vi "RemoteVI Copy Window.vi"(0 "hwnd":u64, 11 "error in":errorcluster) -> (4 "pixmap":u32[][](array[numeric]), 15 "error out":errorcluster)   [LabVIEW 2020, in "RemoteVI.lvlib"]
doc: "Copies the CLIENT AREA of the window hwnd into a 2D U32 pixmap [row, column] of 0x00RRGGBB values as Windows composited it last: user32 GetDC of the window, gdi32 BitBlt (SRCCOPY) into a memory bitmap of the client size (user32 GetClientRect), GetDIBits as 32-bit top-down rows. With desktop composition every top-level window draws into its own surface, so this sees the window's pixels whether or not it is covered by other windows (measured on Windows 11 with a LabVIEW front panel behind a maximised window, pixel-identical to PrintWindow) - and unlike PrintWindow it does not make the window draw itself again: about 2-5 ms for an 817 x 543 panel instead of 40-50 ms with PrintWindow, during which LabVIEW's UI thread repainted the whole window (graph included) for every frame and was busy for nothing else (measured on the demo). A minimized window has an empty client area; pixmap is then empty. No VI Server call, so it works while an open popup holds LabVIEW's UI thread. Every GDI object is deselected and released again, also when an earlier step failed. error out carries error in, a Call Library Function Node error, 5003 when BitBlt failed or 5001 when GetDIBits copied no line."
uses:
  RemoteVI.lvlib
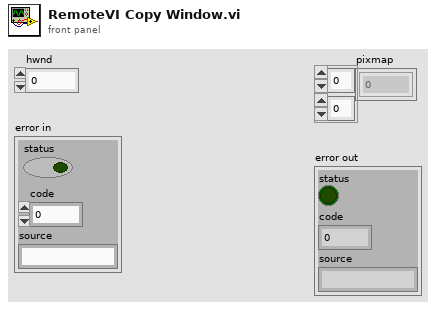
[diagram p1: front panel]
types:
  T1 = cluster{"left":i32, "top":i32, "right":i32, "bottom":i32}
  T2 = cluster{"biSize":u32, "right":i32, i32, "biPlanes":u16, "biBitCount":u16, u32, u32, "zero":i32, "zero":i32, u32, u32, u32}
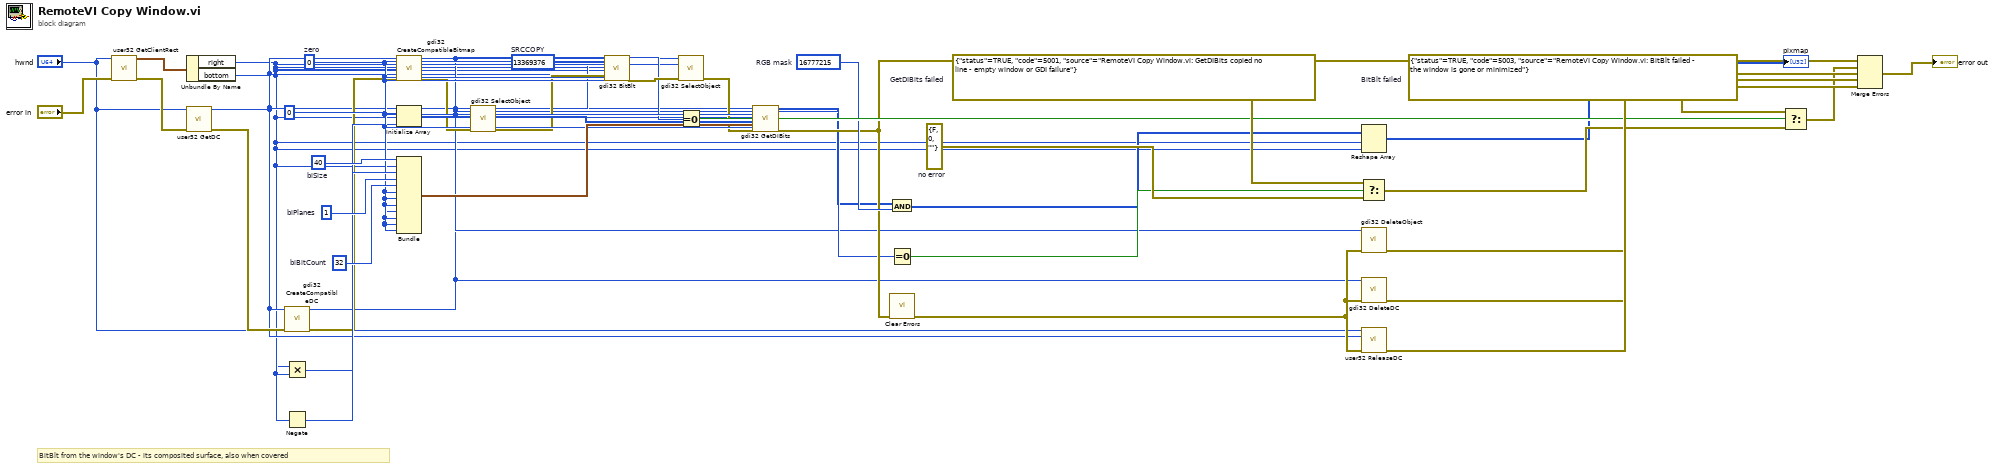
[diagram p0: block diagram]
diagram:
  w39 = errorcluster {"status"=FALSE, "code"=0, "source"=""}  # no error
  w38 = errorcluster {"status"=TRUE, "code"=5001, "source"="RemoteVI Copy Window.vi: GetDIBits copied no line - empty window or GDI failure"}  # GetDIBits failed
  w37 = errorcluster {"status"=TRUE, "code"=5003, "source"="RemoteVI Copy Window.vi: BitBlt failed - the window is gone or minimized"}  # BitBlt failed
  w33 = u32 16777215  # RGB mask
  w28 = u16 32  # biBitCount
  w27 = u16 1  # biPlanes
  w26 = u32 40  # biSize
  w23 = u32 0
  w18 = u32 13369376  # SRCCOPY
  w17 = 0  # zero
  # "BitBlt from the window's DC - its composited surface, also when covered"
  n1 = call "user32 GetClientRect.vi"("hWnd"="hwnd", "error in"="error in") -> ("RECT"=w5:T1, "error out"=w6:errorcluster)  [unwired: 11 in, 1 out]
  n2 = Unbundle By Name(w5) -> ("right"=w7:i32, "bottom"=w8:i32)
  n3 = call "user32 GetDC.vi"("hWnd"="hwnd", "error in"=w6) -> ("HDC"=w9:u64, "error out"=w10:errorcluster)  [unwired: 12 in]
  n4 = call "gdi32 CreateCompatibleDC.vi"("hdc"=w9, "error in"=w10) -> ("HDC"=w11:u64, "error out"=w12:errorcluster)  [unwired: 12 in]
  n5 = Multiply(x=w7, y=w8) -> (x*y=w22:i32)
  n6 = Negate(x=w8) -> (-x=w25:i32)
  n7 = call "gdi32 CreateCompatibleBitmap.vi"("hdc"=w9, "cx"=w7, "cy"=w8, "error in"=w12) -> ("HBITMAP"=w13:u64, "error out"=w14:errorcluster)  [unwired: 10 in]
  n8 = Initialize Array(w23, w22) -> (w24:u32[])
  n9 = Bundle("biSize"=w26, "right"=w7, w25, "biPlanes"=w27, "biBitCount"=w28, w23, w23, "zero"=w17, "zero"=w17, w23, w23, w23) -> (w29:T2)  [unwired: 1 in]
  n10 = call "gdi32 SelectObject.vi"("hdc"=w11, "h"=w13, "error in"=w14) -> ("previous object"=w15:u64, "error out"=w16:errorcluster)  [unwired: 11 in]
  n11 = call "gdi32 BitBlt.vi"("hdc"=w11, "x"=w17, "y"=w17, "cx"=w7, "cy"=w8, "hdcSrc"=w9, "x1"=w17, "y1"=w17, "rop"=w18, "error in"=w16) -> ("return value"=w19:i32, "error out"=w20:errorcluster)  [unwired: 16 in]
  n12 = call "gdi32 SelectObject.vi"("hdc"=w11, "h"=w15, "error in"=w20) -> ("error out"=w21:errorcluster)  [unwired: 11 in, 1 out]
  n13 = Equal To 0?(x=w19) -> (x = 0?=w35:bool)
  n14 = call "gdi32 GetDIBits.vi"("hdc"=w9, "hbm"=w13, "start"=w23, "cLines"=w8, "lpvBits"=w24, "lpbmi"=w29, "usage"=w23, "error in"=w21) -> ("lpvBits out"=w30:u32[], "return value"=w31:i32, "error out"=w32:errorcluster)  [unwired: 17 in]
  n15 = And(x=w30, y=w33) -> (x .and. y?=w34:u32[])
  n16 = Equal To 0?(x=w31) -> (x = 0?=w36:bool)
  n17 = call <vilib>:"Clear Errors.vi"("error in (no error)"=w32) -> ("error out"=w42:errorcluster)  [unwired: 5 in, 1 out]
  n18 = Reshape Array(w34, w8, w7) -> (→"pixmap":u32[][])
  n19 = Select(t=w38, s=w36, f=w39) -> (s? t:f=w40:errorcluster)
  n20 = call "gdi32 DeleteObject.vi"("ho"=w13, "error in"=w42) -> ("error out"=w43:errorcluster)  [unwired: 12 in, 1 out]
  n21 = call "gdi32 DeleteDC.vi"("hdc"=w11, "error in"=w42) -> ("error out"=w44:errorcluster)  [unwired: 12 in, 1 out]
  n22 = call "user32 ReleaseDC.vi"("hWnd"="hwnd", "hDC"=w9, "error in"=w42) -> ("error out"=w45:errorcluster)  [unwired: 11 in, 1 out]
  n23 = Select(t=w37, s=w35, f=w40) -> (s? t:f=w41:errorcluster)
  n24 = Merge Errors(w32, w41, w43, w44, w45) -> (→"error out":errorcluster)
